vi "Fine Timing Synchronization.vi"(9 "Long Preamble":cdb[](array[numeric]), 10 "Coarse packet est":dbl, 11 "Frame after coarse freq sync":cdb[](array[numeric])) -> (2 "Fine packet est":dbl, 3 "Frame after fine time sync":cdb[](array[numeric]))   [LabVIEW 2024]
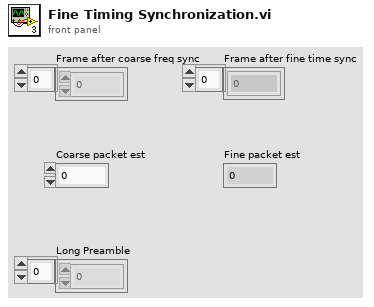
[diagram p1: front panel]
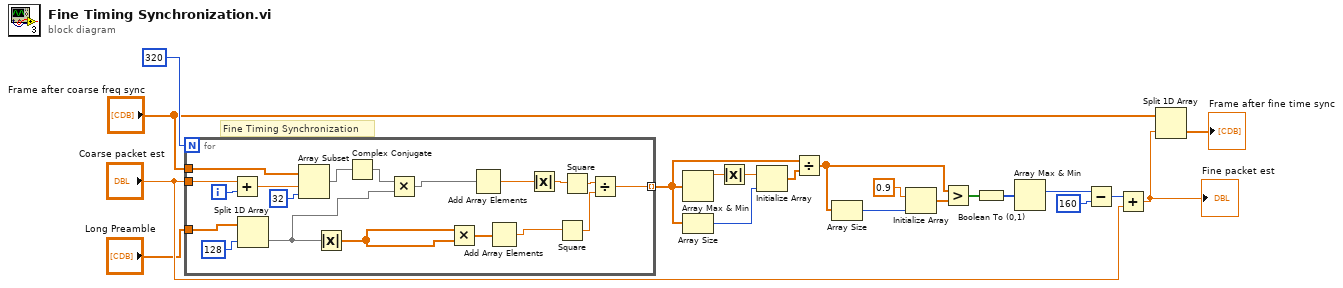
[diagram p0: block diagram]
diagram:
  # "Fine Timing Synchronization"
  n1 = for {
    N: 320 -> [_]
    tunnel: "Long Preamble" -> [w39]
    tunnel: "Frame after coarse freq sync" -> [w33]
    tunnel: [w32] -> w4 mode=indexing
    tunnel: "Coarse packet est" -> [w29]
    i -> [w30]
    n2 = Add(x=w29, y=w30) -> (x+y=w31:dbl)
    n3 = Split 1D Array(array=w39, index=128) -> (second subarray=w25:cdb[])  [unwired: 1 out]
    n4 = Array Subset(array=w33, index=w31, length=32) -> (w21:cdb[])
    n5 = Absolute Value(x=w25) -> (abs(x)=w28:dbl[])
    n6 = Complex Conjugate(1:w21) -> (0:w22:cdb[])
    n7 = Multiply(x=w22, y=w25) -> (x*y=w24:cdb[])
    n8 = Multiply(x=w28, y=w28) -> (x*y=w27:dbl[])
    n9 = Add Array Elements(numeric array=w24) -> (sum=w23:cdb)
    n10 = Add Array Elements(numeric array=w27) -> (sum=w26:dbl)
    n11 = Absolute Value(x=w23) -> (abs(x)=w36:dbl)
    n12 = Square(x=w26) -> (x^2=w35:dbl)
    n13 = Square(x=w36) -> (x^2=w34:dbl)
    n14 = Divide(x=w34, y=w35) -> (x/y=w32:dbl)
  }
  n15 = Array Max & Min(array=w4) -> (max value=w15:dbl)  [unwired: 3 out]
  n16 = Array Size(array=w4) -> (size(s)=w3:i32)
  n17 = Absolute Value(x=w15) -> (abs(x)=w1:dbl)
  n18 = Initialize Array(w1, w3) -> (w2:dbl[])
  n19 = Divide(x=w4, y=w2) -> (x/y=w9:dbl[])
  n20 = Array Size(array=w9) -> (size(s)=w5:i32)
  n21 = Initialize Array(0.9 ("element"), w5) -> (w7:dbl[])
  n22 = Greater?(x=w9, y=w7) -> (0:w8:bool[])
  n23 = Boolean To (0,1)(Boolean=w8) -> (0, 1=w10:i16[])
  n24 = Array Max & Min(array=w10) -> (max index (indices)=w11:i32)  [unwired: 3 out]
  n25 = Subtract(x=w11, y=160) -> (x-y=w17:i32)
  n26 = Add(x=w17, y="Coarse packet est") -> (x+y=w19:dbl)
  "Fine packet est" <- w19
  n27 = Split 1D Array(array="Frame after coarse freq sync", index=w19) -> (second subarray=→"Frame after fine time sync":cdb[])  [unwired: 1 out]
